vi "Create Element.vi"(8 "error in":errorcluster, 9 "Type Definitions Folder":path, 10 "Parameter":T1, 11 "Element Manager in":refnum<class "Element Manager.lvclass">) -> (0 "error out":errorcluster, 2 "IElement":refnum<class "IElement.lvclass">, 3 "Element Manager out":refnum<class "Element Manager.lvclass">)   [LabVIEW 2026, in "Element Manager.lvclass"]
doc: "Create element from function parameter cluster."
uses:
  Element Manager.lvclass
  Type Definitions/Parameter--cluster.ctl
  Interfaces/IElement/IElement.lvclass
  Type Definitions/Data types--enum.ctl
  Type Definitions/Containers--enum.ctl
  Numeric/Numeric.lvclass
  C:/Users/juanj/Documents/hasbun_wood_engineering/github/py2vi/labview/Interfaces/IElement/IElement.lvclass
  Boolean/Boolean.lvclass
  String/String.lvclass
  Cluster/Cluster.lvclass
  Array/Array.lvclass
  C:/Users/juanj/Documents/hasbun_wood_engineering/github/py2vi/labview/Classes/Element/Element.lvclass
  Element/Element.lvclass
  Element Manager.lvclass/Element Manager.ctl
  C:/Users/juanj/Documents/hasbun_wood_engineering/github/py2vi/labview/Classes/Numeric/Numeric.lvclass
  C:/Users/juanj/Documents/hasbun_wood_engineering/github/py2vi/labview/Classes/Boolean/Boolean.lvclass
  C:/Users/juanj/Documents/hasbun_wood_engineering/github/py2vi/labview/Classes/String/String.lvclass
  C:/Users/juanj/Documents/hasbun_wood_engineering/github/py2vi/labview/Classes/Cluster/Cluster.lvclass
  C:/Users/juanj/Documents/hasbun_wood_engineering/github/py2vi/labview/Classes/Array/Array.lvclass
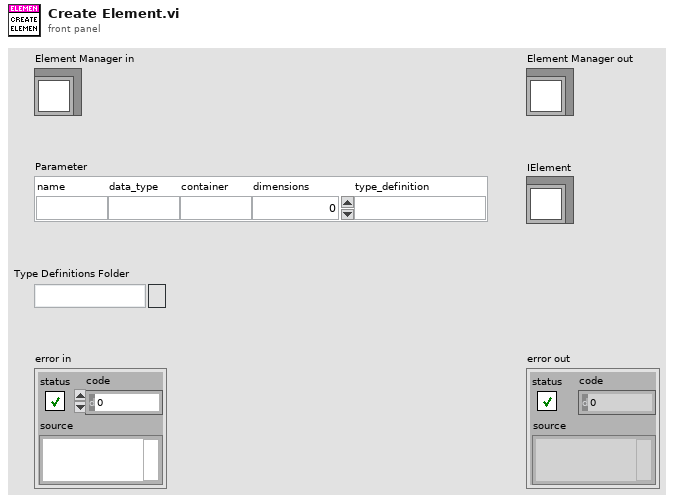
[diagram p1: front panel]
types:
  T1 = typedef "Parameter--cluster.ctl" = cluster{"name":string, "data_type":string, "container":string, "dimensions":i32, "type_definition":string}
  T2 = typedef "Data types--enum.ctl" = enum16{"int", "float", "bool", "str", "TypedDict", "np.bool_", "np.int8", "np.int16", "np.int32", "np.int64", "np.uint8", "np.uint16", "np.uint32", "np.uint64", "np.float32", "np.float64", "np.str_"}
  T3 = typedef "Containers--enum.ctl" = enum16{"", "list", "np.ndarray"}
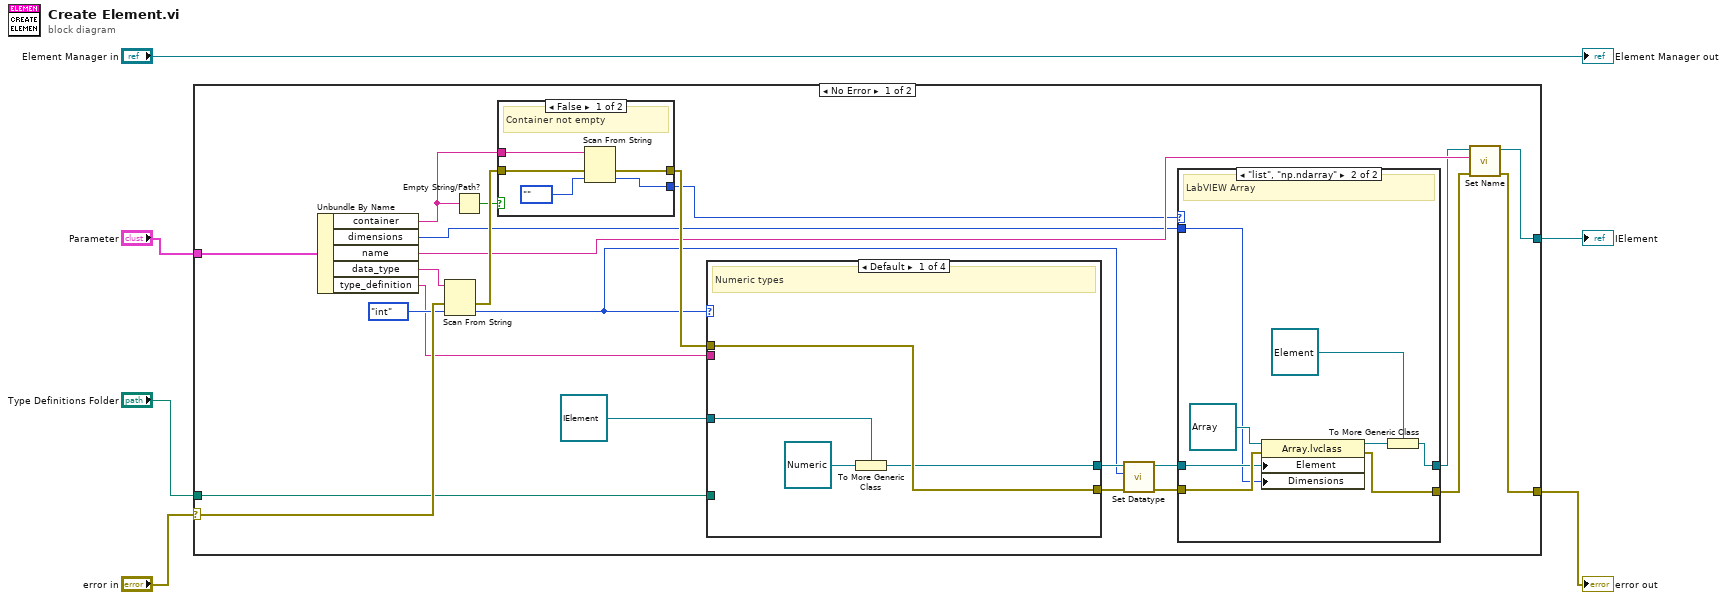
[diagram p0: block diagram]
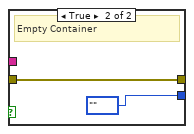
[diagram p2: hidden frame]
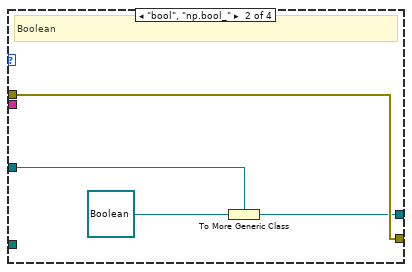
[diagram p4: hidden frame]
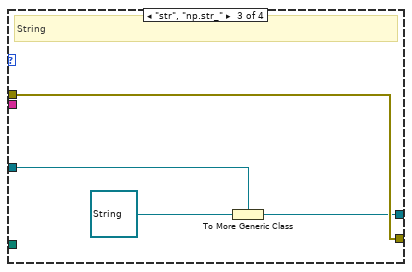
[diagram p5: hidden frame]
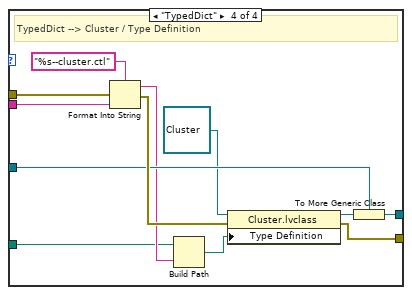
[diagram p6: hidden frame]
diagram:
  n1 = case shown="No Error" "error in" {
    selector: "error in" -> [w26 w71]
    tunnel: "Parameter" -> [w12 _]
    tunnel: "Type Definitions Folder" -> [w11 _]
    tunnel: [w23 w71] -> w5
    tunnel: [w7 _] -> w1
    frame No Error {
      n2 = Unbundle By Name(w12) -> ("container"=w14:string, "dimensions"=w16:i32, "name"=w19:string, "data_type"=w22:string, "type_definition"=w20:string)
      n3 = Scan From String(input string=w22, error in=w26, default 1=Data_types--enum."int" ("Data types")) -> (error out=w28:errorcluster, output 1=w17:T2)  [unwired: 2 in, 2 out]
      n4 = Empty String/Path?(string/path=w14) -> (empty?=w15:bool)
      n5 = case shown="False" w15 {
        tunnel: w14 -> [w31 _]
        tunnel: [w30 Containers--enum."" ("Containers")] -> w13
        tunnel: w28 -> [w34 w36]
        tunnel: [w33 w36] -> w27
        frame False {
          # "Container not empty"
          n6 = Scan From String(input string=w31, error in=w34, default 1=Containers--enum."" ("Containers")) -> (error out=w33:errorcluster, output 1=w30:T3)  [unwired: 2 in, 2 out]
        }
        frame True {
          # "Empty Container"
        }
      }
      n7 = case shown="Default" w17 {
        tunnel: refnum<class "IElement.lvclass"> refnum ("IElement.lvclass") -> [w48 w52 w57 w67]
        tunnel: [w47 w53 w56 w65] -> w18
        tunnel: w11 -> [_ _ _ w61]
        tunnel: w20 -> [_ _ _ w59]
        tunnel: w27 -> [w50 w54 w58 w70]
        tunnel: [w50 w54 w58 w68] -> w29
        frame Default {
          # "Numeric types"
          n8 = To More Generic Class(target class=w48, reference=refnum<class "Numeric.lvclass"> refnum ("Numeric.lvclass")) -> (generic class reference=w47:refnum<class "IElement.lvclass">)
        }
        frame "bool", "np.bool_" {
          # "Boolean"
          n9 = To More Generic Class(target class=w52, reference=refnum<class "Boolean.lvclass"> refnum ("Boolean.lvclass")) -> (generic class reference=w53:refnum<class "IElement.lvclass">)
        }
        frame "str", "np.str_" {
          # "String"
          n10 = To More Generic Class(target class=w57, reference=refnum<class "String.lvclass"> refnum ("String.lvclass")) -> (generic class reference=w56:refnum<class "IElement.lvclass">)
        }
        frame "TypedDict" {
          # "TypedDict --> Cluster / Type Definition"
          n11 = Format Into String(format string="%s--cluster.ctl", error in=w70, w59) -> (resulting string=w63:string, error out=w69:errorcluster)  [unwired: 1 in]
          n12 = Build Path(base path=w61, name or relative path=w63) -> (appended path=w60:path)
          n13 = property class="Cluster.lvclass"(reference=refnum<class "Cluster.lvclass"> refnum ("Cluster.lvclass"), error in=w69, "Type Definition"=w60) -> (reference out=w64:refnum<class "Cluster.lvclass">, error out=w68:errorcluster)
          n14 = To More Generic Class(target class=w67, reference=w64) -> (generic class reference=w65:refnum<class "IElement.lvclass">)
        }
      }
      n15 = call-dynamic "Set Datatype.vi"("error in"=w29, "Datatype"=w17, "IElement in"=w18) -> ("error out"=w25:errorcluster, "IElement out"=w9:refnum<class "IElement.lvclass">)  [unwired: 7 in]
      n16 = case shown="\"list\", \"np.ndarray\"" w13 {
        tunnel: w9 -> [w37 w43]
        tunnel: w16 -> [_ w42]
        tunnel: [w37 w39] -> w8
        tunnel: w25 -> [w38 w46]
        tunnel: [w38 w45] -> w24
        frame Default {
          # "Scalar"
        }
        frame "list", "np.ndarray" {
          # "LabVIEW Array"
          n17 = property class="Array.lvclass"(reference=refnum<class "Array.lvclass"> refnum ("Array.lvclass"), error in=w46, "Element"=w43, "Dimensions"=w42) -> (reference out=w41:refnum<class "Array.lvclass">, error out=w45:errorcluster)
          n18 = To More Generic Class(target class=refnum<class "Element.lvclass"> refnum ("Element.lvclass"), reference=w41) -> (generic class reference=w39:refnum<class "Element.lvclass">)
        }
      }
      n19 = call-dynamic "Set Name.vi"("error in"=w24, "Name"=w19, "IElement in"=w8) -> ("error out"=w23:errorcluster, "IElement out"=w7:refnum<class "IElement.lvclass">)  [unwired: 7 in]
    }
    frame Error {
      # "Pass error without further action."
    }
  }
  "error out" <- w5
  "IElement" <- w1
  "Element Manager out" <- "Element Manager in"
